vi "Get Menu Labels.vi"(8 "error in":errorcluster, 11 "Menu":T2) -> (0 "error out":errorcluster, 2 "Right Menu":T1, 3 "Left Menu":T1)   [LabVIEW 2026]
doc: "Takes a menu (ATM Menu.ctl) and returns the button labels of its Left and Right side as the two string clusters the ATM front panel shows beside the function buttons (Left Menu and Right Menu). Element order is Item 1, Item 2, Item 3, top to bottom, so the outputs wire straight into the front-panel indicators.\n\nError behaviour: error in is passed to error out unchanged; the labels are returned in every case."
uses:
  Controls/ATM States.ctl
  Controls/ATM Menu Item.ctl
  Controls/ATM Menu Side.ctl
  Controls/ATM Menu.ctl
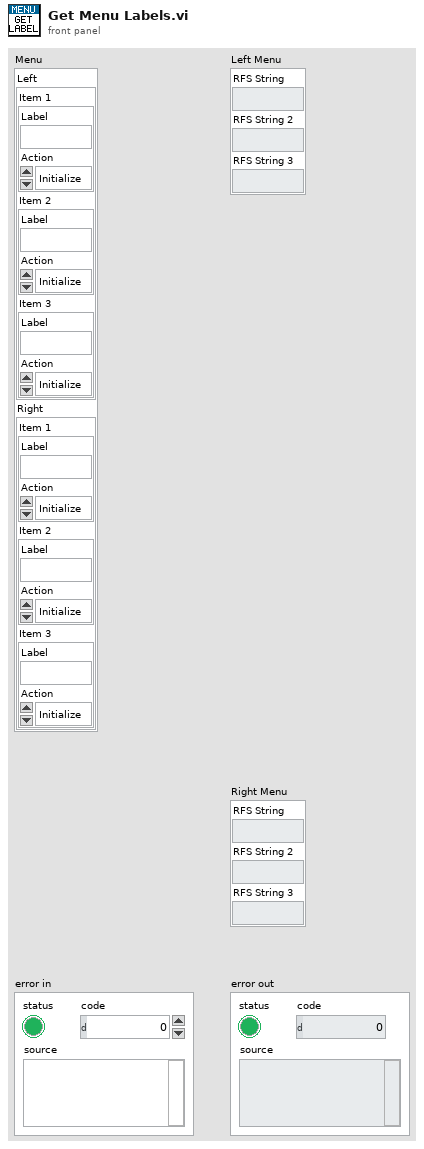
[diagram p1: front panel]
types:
  T1 = cluster{"RFS String":string, "RFS String 2":string, "RFS String 3":string}
  T2 = typedef "ATM Menu.ctl" = cluster{"Left":T3, "Right":T3}
  T3 = typedef "ATM Menu Side.ctl" = cluster{"Item 1":T4, "Item 2":T4, "Item 3":T4}
  T4 = typedef "ATM Menu Item.ctl" = cluster{"Label":string, "Action":T5}
  T5 = typedef "ATM States.ctl" = enum16{"Initialize", "Wait for Event", "Card Inserted", "Process Input", "Verify Account", "Show Main Menu", "Deposit Prompt", "Withdraw Prompt", "Deposit", "Withdraw", "Fast Cash", "Balance Inquiry", "None", "Terminate Session", "Exit"}
  T6 = cluster{"Label":string, "Label":string, "Label":string}
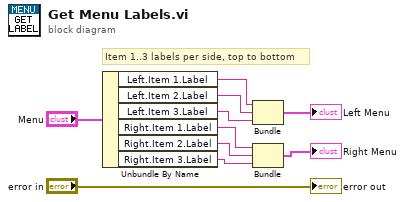
[diagram p0: block diagram]
diagram:
  # "Item 1..3 labels per side, top to bottom"
  n1 = Unbundle By Name("Menu") -> ("Left.Item 1.Label"=w9:string, "Left.Item 2.Label"=w8:string, "Left.Item 3.Label"=w7:string, "Right.Item 1.Label"=w6:string, "Right.Item 2.Label"=w5:string, "Right.Item 3.Label"=w4:string)
  n2 = Bundle("Label"=w9, "Label"=w8, "Label"=w7) -> (→"Left Menu":T6)  [unwired: 1 in]
  n3 = Bundle("Label"=w6, "Label"=w5, "Label"=w4) -> (→"Right Menu":T6)  [unwired: 1 in]
  "error out" <- "error in"
